vi "Process TDMS Metadata.vi"(0 "Sift TDMS Uploader in":refnum<class "Sift TDMS Uploader.lvclass">, 1 "TDMS File":path, 3 "error in (no error)":errorcluster) -> (7 "Sift TDMS Uploader out":refnum<class "Sift TDMS Uploader.lvclass">, 8 "Metadata":map{string, variant}(c390), 10 "error out":errorcluster)   [LabVIEW 2024, in "Sift TDMS Uploader.lvlib" / "Sift TDMS Uploader.lvclass"]
doc: "Parses and returns the updated TDMS file metadata using the configuration file."
uses:
  Sift TDMS Uploader.lvclass
  Sift TDMS Uploader.lvclass/Sift TDMS Uploader.ctl
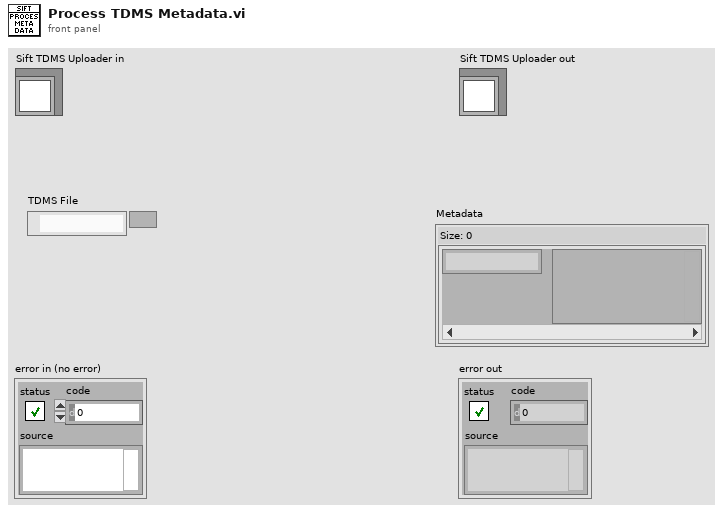
[diagram p1: front panel]
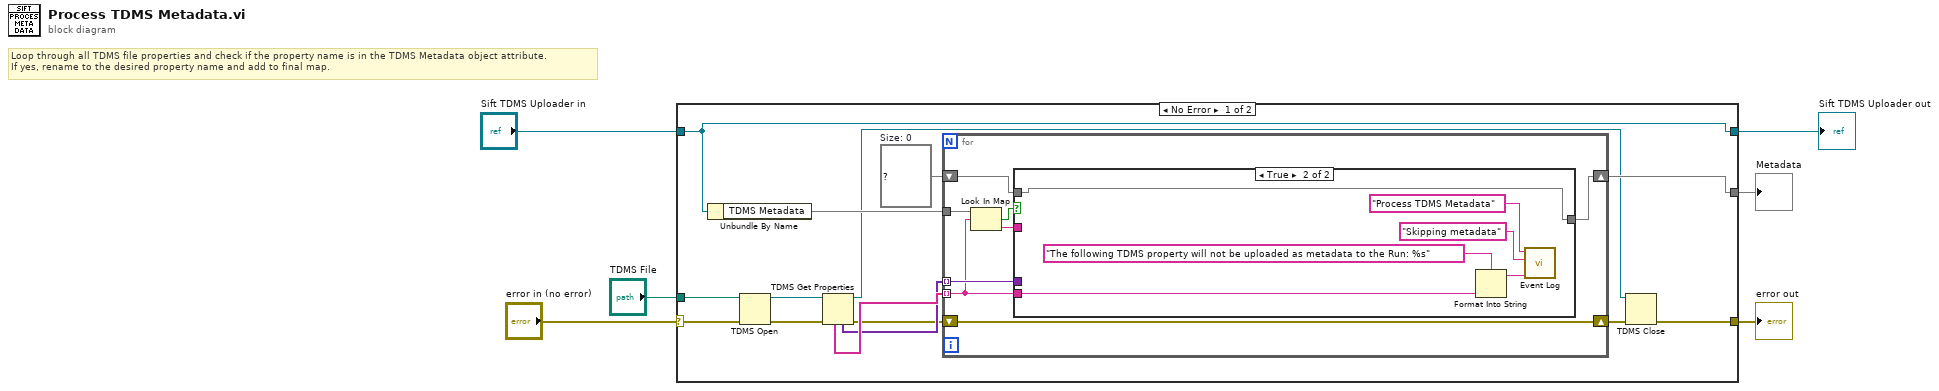
[diagram p0: block diagram]
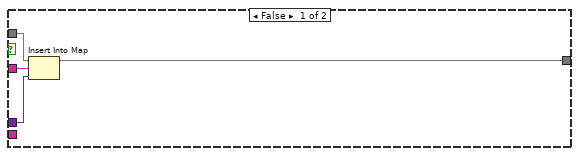
[diagram p2: hidden frame]
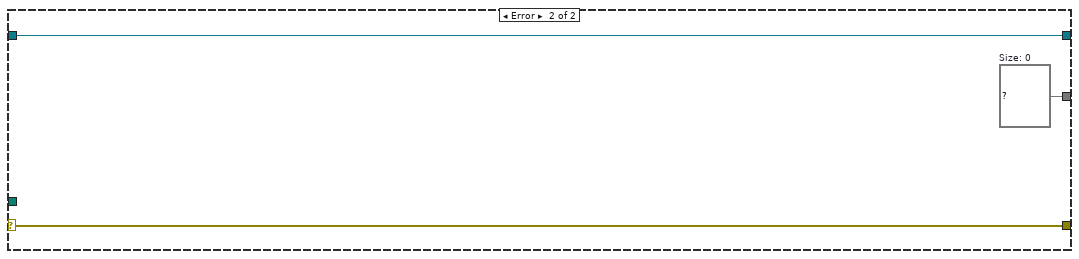
[diagram p3: hidden frame]
diagram:
  # "Loop through all TDMS file properties and check if the property name is in the TDMS Metadata object attribute.\nIf yes, rename to the desired property name and add to final map."
  n1 = case shown="No Error" "error in (no error)" {
    selector: "error in (no error)" -> [w19 w41]
    tunnel: [w9 w41] -> w5
    tunnel: [w16 w40] -> w3
    tunnel: "Sift TDMS Uploader in" -> [w16 w40]
    tunnel: "TDMS File" -> [w20 _]
    tunnel: [w12 w39] -> w1
    frame No Error {
      w8 = map{string, variant} {}  # Size: 0
      n2 = Unbundle By Name(w16) -> ("TDMS Metadata"=w15:map{string, string})
      n3 = TDMS Open(8:w19, 11:w20) -> (0:w17:errorcluster, 3:w18:refnum<k34>)  [unwired: 5 in]
      n4 = TDMS Get Properties(8:w17, 11:w18) -> (0:w11:errorcluster, 3:w7:refnum<k34>, 4:w13:variant[], 6:w14:string[])  [unwired: 4 in, 2 out]
      n5 = for {
        tunnel: w14 -> [w21] mode=indexing
        tunnel: w13 -> [w22] mode=indexing
        shift-right: [w24] -> w10
        shift-left: w11 -> [w24]
        tunnel: w15 -> [w27]
        shift-right: [w26] -> w12
        shift-left: w8 -> [w23]
        n6 = Look In Map(map=w27, key=w21) -> (key not found?=w28:bool, value=w25:string)  [unwired: 1 in]
        n7 = case shown="True" w28 {
          tunnel: w23 -> [w32 w38]
          tunnel: [w31 w38] -> w26
          tunnel: w25 -> [w30 _]
          tunnel: w22 -> [w29 _]
          tunnel: w21 -> [_ w35]
          frame False {
            n8 = Insert Into Map(map in=w32, key=w30, value=w29) -> (map out=w31:map{string, variant})  [unwired: 2 out]
          }
          frame True {
            n9 = Format Into String(format string="The following TDMS property will not be uploaded as metadata to the Run: %s", w35) -> (resulting string=w33:string)  [unwired: 2 in, 1 out]
            n10 = call "Event Log.vi"("Message"=w33, "Event Type"="Skipping metadata", "Location"="Process TDMS Metadata") -> ()  [unwired: 9 in]
          }
        }
      }
      n11 = TDMS Close(8:w10, 11:w7) -> (0:w9:errorcluster)  [unwired: 1 out]
    }
    frame Error {
      w39 = map{string, variant} {}  # Size: 0
    }
  }
  "error out" <- w5
  "Sift TDMS Uploader out" <- w3
  "Metadata" <- w1
